vi "Initialize Game.vi"(10 "height":u32, 11 "width":u32) -> (3 "living cells":bool[][](array[boolean]))   [LabVIEW 2021, in "Game of Life.lvlib"]
doc: "This VI generates a 2D boolean array of living cells in a random fashion with 30% living cell rate."
uses:
  Game of Life.lvlib
  <vilib>/numeric/Random Number (Range) U64.vi
  <vilib>/numeric/sub_Random U32.vi
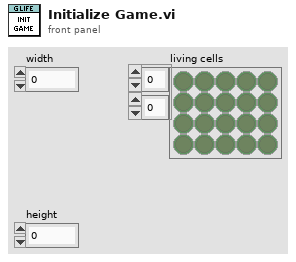
[diagram p1: front panel]
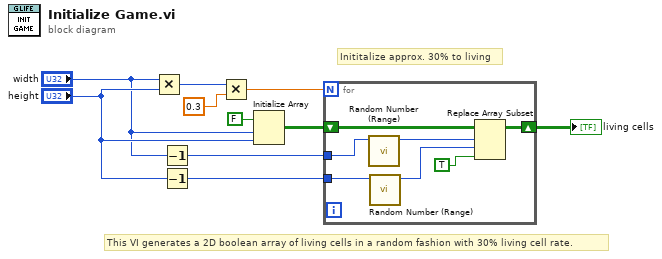
[diagram p0: block diagram]
diagram:
  # "This VI generates a 2D boolean array of living cells in a random fashion with 30% living cell rate."
  # "Inititalize approx. 30% to living"
  n1 = Multiply(x="width", y="height") -> (x*y=w7:u32)
  n2 = Decrement(x="width") -> (x-1=w4:u32)
  n3 = Decrement(x="height") -> (x-1=w5:u32)
  n4 = Multiply(x=w7, y=0.3) -> (x*y=w1:dbl)
  n5 = Initialize Array(FALSE, "width", "height") -> (w6:bool[][])
  n6 = for {
    N: w1 -> [_]
    tunnel: w4 -> [w17]
    tunnel: w5 -> [w16]
    shift-right: [w11] -> w8
    shift-left: w6 -> [w15]
    n7 = call-poly <vilib>:"Random Number (Range).vi"("upper bound (100)"=w17) -> ("number"=w14:u64)  [unwired: 10 in]
    n8 = call-poly <vilib>:"Random Number (Range).vi"("upper bound (100)"=w16) -> ("number"=w13:u64)  [unwired: 10 in]
    n9 = Replace Array Subset(array=w15, new element=TRUE ("new element/subarray"), index (row)=w14, index (col)=w13) -> (w11:bool[][])
  }
  "living cells" <- w8
